vi "Start Triggered Acq.vi"(8 "error in (no error)":errorcluster, 9 "Write to disk?":bool, 10 "Repeat?":bool=TRUE, 11 "DAQ Timed SPIM in":refnum<class "DAQ Timed SPIM.lvclass">) -> (0 "error out":errorcluster, 3 "DAQ Timed SPIM out":refnum<class "DAQ Timed SPIM.lvclass">)   [LabVIEW 2020, in "DAQ Timed SPIM.lvlib" / "DAQ Timed SPIM.lvclass"]
uses:
  DAQ Timed SPIM.lvclass
  C:/Program Files/National Instruments/LabVIEW 2020/vi.lib/ActorFramework/Actor/Actor.lvclass
  DAQ Timed SPIM.lvclass/DAQ Timed SPIM.ctl
  Abstract DAQ Triggered Actor Messages/Start Acq Msg/Start Acq Msg.lvclass/Start Acq Msg.ctl
  <vilib>/ActorFramework/Reply Msg/Reply Msg.lvclass/Reply Msg.ctl
  <vilib>/ActorFramework/Message Enqueuer/Message Enqueuer.lvclass/Message Enqueuer.ctl
  <vilib>/ActorFramework/Actor/Actor.lvclass/Actor.ctl
  DAQ Timed SPIM Messages/Run Main Loop Msg/Run Main Loop Msg.lvclass/Run Main Loop Msg.ctl
  <vilib>/DAQmx/write.llb/DAQmx Write (Digital 2D U8 NChan NSamp).vi
  <vilib>/DAQmx/write.llb/DAQmx Write (Analog 2D DBL NChan NSamp).vi
  <vilib>/ActorFramework/Reply Msg/Send Message And Wait For Response.vi
  <vilib>/ActorFramework/Message Enqueuer/Init from Existing Queue.vi
  <vilib>/ActorFramework/Message Enqueuer/Enqueue.vi
  Abstract DAQ Triggered Actor Messages/Start Acq Msg/Start Acq Msg.lvclass
  C:/Program Files/National Instruments/LabVIEW 2020/vi.lib/ActorFramework/Reply Msg/Reply Msg.lvclass
  <vilib>/ActorFramework/Reply Msg/Reply Msg.lvclass
  C:/Program Files/National Instruments/LabVIEW 2020/vi.lib/ActorFramework/Message/Message.lvclass
  DAQ Timed SPIM Messages/Run Main Loop Msg/Run Main Loop Msg.lvclass
  <vilib>/ActorFramework/Message Priority Queue/Priority Enqueue.vi
  <vilib>/DAQmx/miscellaneous.llb/DAQmx Fill In Error Info.vi
  <vilib>/ActorFramework/Message Enqueuer/Message Enqueuer.lvclass
  <vilib>/ActorFramework/Actor/Actor.lvclass
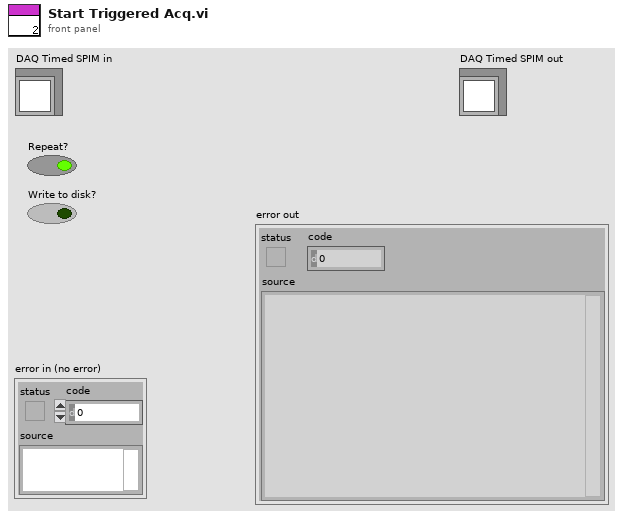
[diagram p1: front panel]
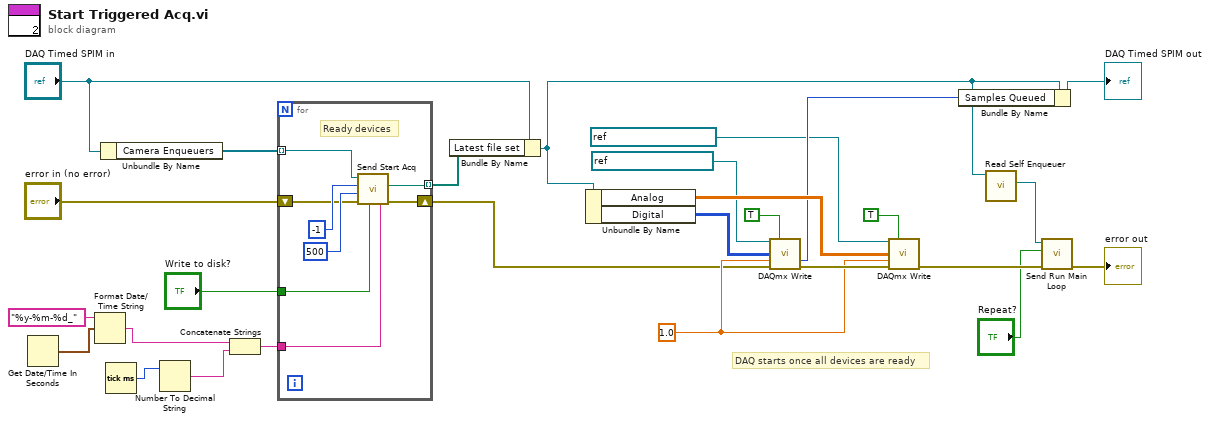
[diagram p0: block diagram]
diagram:
  w13 = 1.0 ("timeout")
  # "DAQ starts once all devices are ready"
  n1 = Get Date/Time In Seconds() -> (seconds since 1Jan1904=w24:timestamp)
  n2 = Format Date/Time String(time format string (%c)="%y-%m-%d_", seconds (now)=w24) -> (date/time string=w22:string)  [unwired: 1 in]
  n3 = Unbundle By Name("DAQ Timed SPIM in") -> ("Camera Enqueuers"=w27:refnum<class "Message Enqueuer.lvclass">[])
  n4 = Tick Count (ms)() -> (millisecond timer value=w23:u32)
  n5 = Number To Decimal String(number=w23) -> (decimal integer string=w21:string)  [unwired: 1 in]
  n6 = Concatenate Strings(w22, w21) -> (w17:string)
  n7 = for {
    tunnel: w27 -> [w35] mode=indexing
    shift-right: [w34] -> w1
    shift-left: "error in (no error)" -> [w31]
    tunnel: [w30] -> w19 mode=indexing
    tunnel: "Write to disk?" -> [w29]
    tunnel: w17 -> [w28]
    # "Ready devices"
    n8 = call "Send Start Acq.vi"("Filename"=w28, "Write to disk"=w29, "error in (no error)"=w31, "timeout in ms (-1)"=500, "Frame Count"=-1, "Message Enqueuer"=w35) -> ("error out"=w34:errorcluster, "File path"=w30:path)  [unwired: 2 in, 2 out]
  }
  n9 = Bundle By Name(cluster="DAQ Timed SPIM in", "Latest file set"=w19) -> (w4:refnum<class "DAQ Timed SPIM.lvclass">)
  n10 = Unbundle By Name(w4) -> ("Analog"=w6:dbl[][], "Digital"=w12:u8[][])
  n11 = call-poly <vilib>:"DAQmx Write.vi"("task/channels in"=refnum<k21> "SPIM_Digital_Task", "auto start"=TRUE, "data"=w12, "timeout"=w13, "error in"=w1) -> ("number of samples written per channel"=w5:u32, "error out"=w14:errorcluster)  [unwired: 8 in, 1 out]
  n12 = call-poly <vilib>:"DAQmx Write.vi"("task/channels in"=refnum<k21> "SPIM_Analog_Task", "auto start"=TRUE, "data"=w6, "timeout"=w13, "error in"=w14) -> ("error out"=w11:errorcluster)  [unwired: 8 in, 2 out]
  n13 = Bundle By Name(cluster=w4, "Samples Queued"=w5) -> (→"DAQ Timed SPIM out":refnum<class "DAQ Timed SPIM.lvclass">)
  n14 = call <vilib>:"Read Self Enqueuer.vi"("Actor"=w4) -> ("Self Enqueuer"=w9:refnum<class "Message Enqueuer.lvclass">)  [unwired: 10 in]
  n15 = call "Send Run Main Loop.vi"("error in (no error)"=w11, "Repeat?"="Repeat?", "Message Enqueuer"=w9) -> ("error out"=→"error out":errorcluster)  [unwired: 7 in, 1 out]
